vi "Reg select run.vi"() -> (2 "Noms sélect run":cluster{"Noms voies sélect run 1COM":string[]}[](array[cluster]), 3 "Adresses sélect run":cluster{"Adresses run 1COM reg":u8[]}[](array[cluster]), 4 "COM run":refnum<visa-resource-name>[](array[refnum]))   [LabVIEW 2022 SP3]
uses:
  Variables globales/Variables glob EUROTHERM.vi
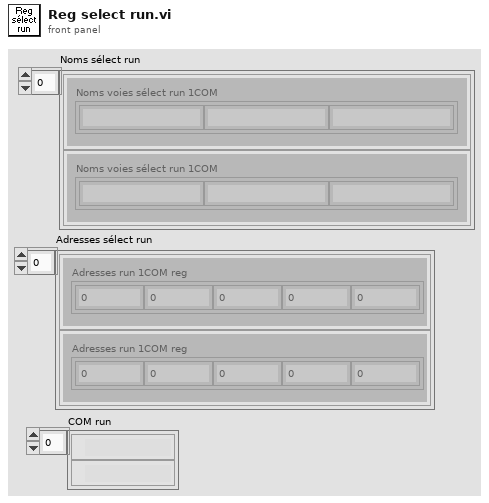
[diagram p1: front panel]
types:
  T1 = cluster{"Noms voies select acqui 1COM":string[]}[]
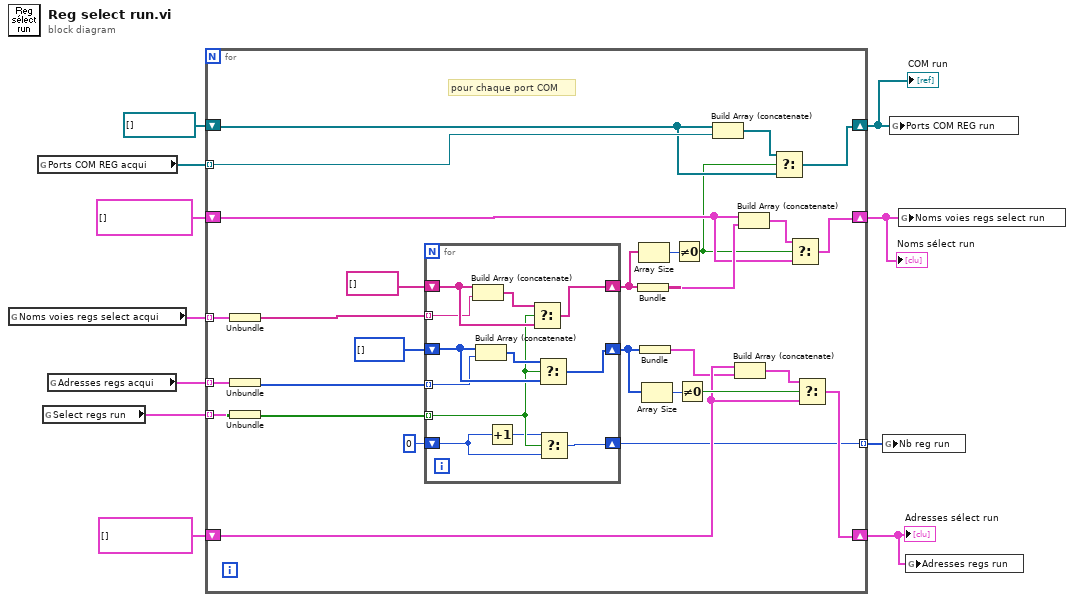
[diagram p0: block diagram]
diagram:
  n1 = global read "Variables glob EUROTHERM.vi" "Noms voies regs select acqui"() -> (w11:T1)
  n2 = global read "Variables glob EUROTHERM.vi" "Ports COM REG acqui"() -> (w4:refnum<visa-resource-name>[])
  n3 = global read "Variables glob EUROTHERM.vi" "Select regs run"() -> (w9:cluster{"Sélect run 1COM reg":bool[]}[])
  n4 = global read "Variables glob EUROTHERM.vi" "Adresses regs acqui"() -> (w10:cluster{"Adresses acqui 1COM reg":u16[]}[])
  n5 = for {
    tunnel: w11 -> [w34] mode=indexing
    tunnel: w10 -> [w33] mode=indexing
    tunnel: w9 -> [w32] mode=indexing
    shift-right: [w26] -> w8
    shift-left: cluster{string[]}[] [] -> [w27]
    shift-right: [w19] -> w7
    shift-left: cluster{u16[]}[] [] -> [w21]
    tunnel: w4 -> [w17] mode=indexing
    shift-right: [w16] -> w3
    shift-left: refnum<visa-resource-name>[] [] -> [w15]
    tunnel: [w13] -> w1 mode=indexing
    # "pour chaque port COM"
    n6 = Unbundle(w34) -> ("Noms voies select acqui 1COM"=w37:string[])
    n7 = Unbundle(w33) -> ("Adresses acqui 1COM reg"=w36:u16[])
    n8 = Unbundle(w32) -> ("Sélect run 1COM reg"=w35:bool[])
    n9 = for {
      tunnel: w37 -> [w45] mode=indexing
      tunnel: w35 -> [w43] mode=indexing
      shift-right: [w49] -> w22
      shift-left: u8[] [] -> [w46]
      shift-right: [w48] -> w31
      shift-left: string[] [] -> [w47]
      tunnel: w36 -> [w44] mode=indexing
      shift-right: [w40] -> w13
      shift-left: u8 0 -> [w41]
      n10 = Build Array (concatenate)(w47, w45) -> (w51:string[])
      n11 = Build Array (concatenate)(w46, w44) -> (w50:u16[])
      n12 = Increment(x=w41) -> (x+1=w42:u8)
      n13 = Select(t=w51, s=w43, f=w47) -> (s? t:f=w48:string[])
      n14 = Select(t=w50, s=w43, f=w46) -> (s? t:f=w49:u16[])
      n15 = Select(t=w42, s=w43, f=w41) -> (s? t:f=w40:u8)
    }
    n16 = Bundle(w31) -> (w29:cluster{string[]})  [unwired: 1 in]
    n17 = Array Size(array=w31) -> (size(s)=w30:i32)
    n18 = Bundle(w22) -> (w20:cluster{u16[]})  [unwired: 1 in]
    n19 = Array Size(array=w22) -> (size(s)=w23:i32)
    n20 = Not Equal To 0?(x=w30) -> (x != 0?=w14:bool)
    n21 = Not Equal To 0?(x=w23) -> (x != 0?=w24:bool)
    n22 = Build Array (concatenate)(w15, w17) -> (w18:refnum<visa-resource-name>[])
    n23 = Build Array (concatenate)(w21, w20) -> (w25:cluster{u16[]}[])
    n24 = Build Array (concatenate)(w27, w29) -> (w28:cluster{string[]}[])
    n25 = Select(t=w18, s=w14, f=w15) -> (s? t:f=w16:refnum<visa-resource-name>[])
    n26 = Select(t=w28, s=w14, f=w27) -> (s? t:f=w26:cluster{string[]}[])
    n27 = Select(t=w25, s=w24, f=w21) -> (s? t:f=w19:cluster{u16[]}[])
  }
  "Noms sélect run" <- w8
  "Adresses sélect run" <- w7
  "COM run" <- w3
  n28 = global write "Variables glob EUROTHERM.vi" "Nb reg run"(w1) -> ()
  n29 = global write "Variables glob EUROTHERM.vi" "Ports COM REG run"(w3) -> ()
  n30 = global write "Variables glob EUROTHERM.vi" "Noms voies regs select run"(w8) -> ()
  n31 = global write "Variables glob EUROTHERM.vi" "Adresses regs run"(w7) -> ()
